vi "JUnit Aggregate.vi"() -> ()   [LabVIEW 2013]
doc: "This example illustrates how multiple test suites can be combined in one aggregate JUnit XML report."
uses:
  JUnit XML/Test Suites/Test Suites.lvclass
  JUnit XML/Test Case/Test Case.lvclass
  JUnit XML/Test Suite/Test Suite.lvclass
panel:
  out "XML":string
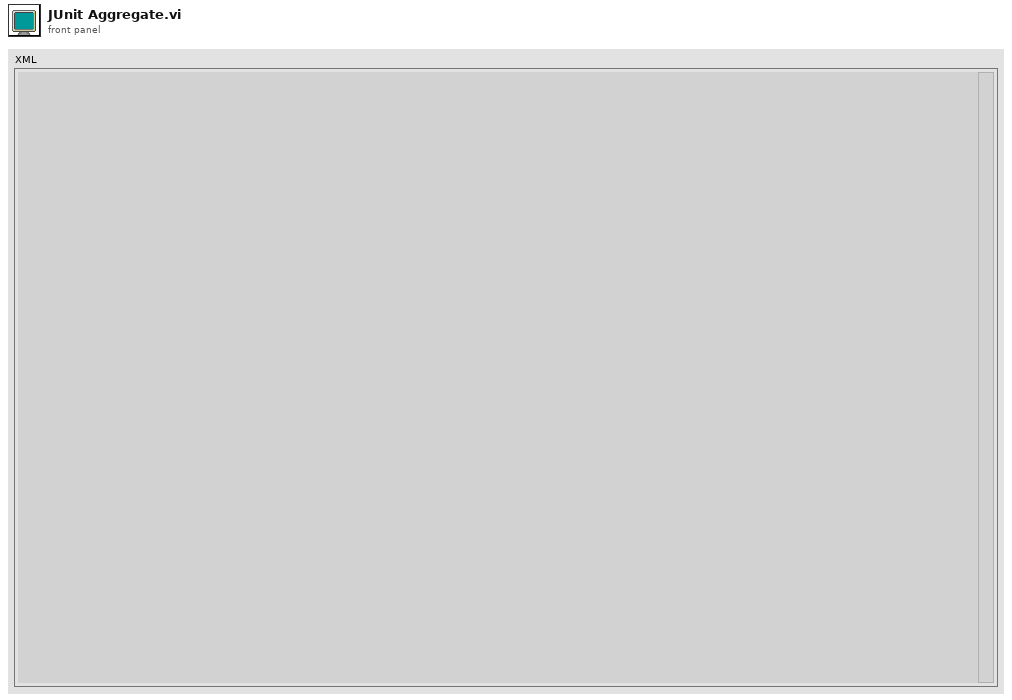
[diagram p1: front panel]
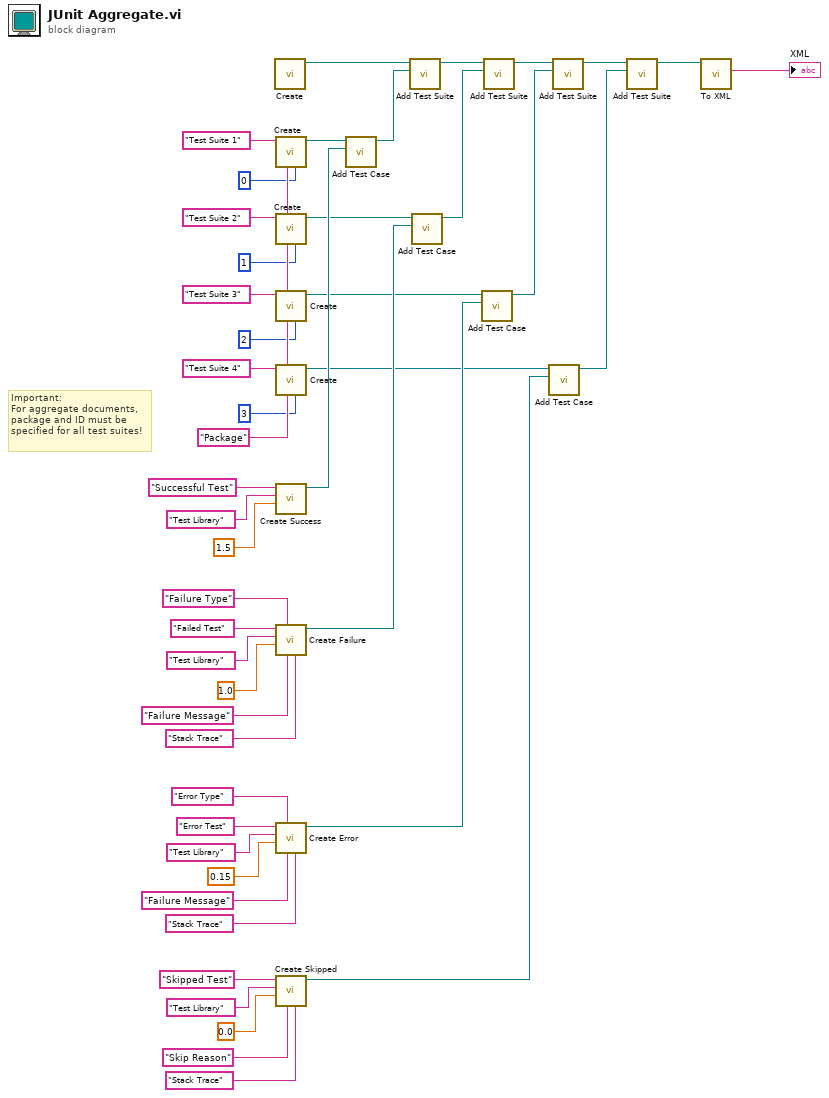
[diagram p0: block diagram]
diagram:
  w5 = "Package" ("Package (\"\" = undefined)")
  # "Important:\nFor aggregate documents,\npackage and ID must be\nspecified for all test suites!"
  n1 = call "Create.vi"() -> ("Test Suites"=w20:refnum<class "Test Suites.lvclass">)  [unwired: 10 in, 1 out]
  n2 = call "Create.vi"("Id (-1 = undefined)"=0, "Package (\"\" = undefined)"=w5, "Name"="Test Suite 1") -> ("Test Suite"=w42:refnum<class "Test Suite.lvclass">)  [unwired: 7 in, 1 out]
  n3 = call "Create.vi"("Id (-1 = undefined)"=1, "Package (\"\" = undefined)"=w5, "Name"="Test Suite 2") -> ("Test Suite"=w15:refnum<class "Test Suite.lvclass">)  [unwired: 7 in, 1 out]
  n4 = call "Create.vi"("Id (-1 = undefined)"=2, "Package (\"\" = undefined)"=w5, "Name"="Test Suite 3") -> ("Test Suite"=w14:refnum<class "Test Suite.lvclass">)  [unwired: 7 in, 1 out]
  n5 = call "Create.vi"("Id (-1 = undefined)"=3, "Package (\"\" = undefined)"=w5, "Name"="Test Suite 4") -> ("Test Suite"=w13:refnum<class "Test Suite.lvclass">)  [unwired: 7 in, 1 out]
  n6 = call "Create Success.vi"("Time"=1.5, "Classname"="Test Library", "Name"="Successful Test") -> ("Test Case"=w41:refnum<class "Test Case.lvclass">)  [unwired: 7 in, 1 out]
  n7 = call "Create Failure.vi"("Stack Trace"="Stack Trace", "Message"="Failure Message", "Type"="Failure Type", "Time"=1.0, "Classname"="Test Library", "Name"="Failed Test") -> ("Test Case"=w34:refnum<class "Test Case.lvclass">)  [unwired: 4 in, 1 out]
  n8 = call "Create Error.vi"("Stack Trace"="Stack Trace", "Message"="Failure Message", "Type"="Error Type", "Time"=0.15, "Classname"="Test Library", "Name"="Error Test") -> ("Test Case"=w27:refnum<class "Test Case.lvclass">)  [unwired: 4 in, 1 out]
  n9 = call "Create Skipped.vi"("Stack Trace"="Stack Trace", "Message"="Skip Reason", "Time"=0.0, "Classname"="Test Library", "Name"="Skipped Test") -> ("Test Case"=w21:refnum<class "Test Case.lvclass">)  [unwired: 5 in, 1 out]
  n10 = call "Add Test Case.vi"("Test Case"=w41, "Test Suite in"=w42) -> ("Test Suite out"=w19:refnum<class "Test Suite.lvclass">)  [unwired: 8 in, 1 out]
  n11 = call "Add Test Suite.vi"("Test Suite"=w19, "Test Suites in"=w20) -> ("Test Suites out"=w12:refnum<class "Test Suites.lvclass">)  [unwired: 8 in, 1 out]
  n12 = call "Add Test Case.vi"("Test Case"=w34, "Test Suite in"=w15) -> ("Test Suite out"=w11:refnum<class "Test Suite.lvclass">)  [unwired: 8 in, 1 out]
  n13 = call "Add Test Case.vi"("Test Case"=w27, "Test Suite in"=w14) -> ("Test Suite out"=w10:refnum<class "Test Suite.lvclass">)  [unwired: 8 in, 1 out]
  n14 = call "Add Test Suite.vi"("Test Suite"=w11, "Test Suites in"=w12) -> ("Test Suites out"=w9:refnum<class "Test Suites.lvclass">)  [unwired: 8 in, 1 out]
  n15 = call "Add Test Case.vi"("Test Case"=w21, "Test Suite in"=w13) -> ("Test Suite out"=w8:refnum<class "Test Suite.lvclass">)  [unwired: 8 in, 1 out]
  n16 = call "Add Test Suite.vi"("Test Suite"=w10, "Test Suites in"=w9) -> ("Test Suites out"=w7:refnum<class "Test Suites.lvclass">)  [unwired: 8 in, 1 out]
  n17 = call "Add Test Suite.vi"("Test Suite"=w8, "Test Suites in"=w7) -> ("Test Suites out"=w6:refnum<class "Test Suites.lvclass">)  [unwired: 8 in, 1 out]
  n18 = call-dynamic "To XML.vi"("Serializable in"=w6) -> ("XML"=→"XML":string)  [unwired: 9 in, 1 out]
